vi "Reverse_PolarityTest.vi"(8 "error in (no error)":errorcluster) -> (0 "error out":errorcluster)   [LabVIEW 2025]
uses:
  SubVIs/All test cluster.ctl
  SubVIs/All_enum_ctl.ctl
  SubVIs/Arduino_lamps.ctl
  SubVIs/Lamps_global.vi
  <vilib>/Utility/file.llb/Write Delimited Spreadsheet (string).vi
  <instrlib>/BK Precision 9200 Series/BK Precision 9200 Series.lvlib
  <instrlib>/Keithley 2260B/Keithley 2260B.lvlib
panel:
  out "Table 2":string[][](table)
  in  "ESP PORT":refnum<visa-resource-name>
  out "Connected? 2":bool caption="Long Blank Button"
  out "Tick Time(s)":dbl
  out "Status":string
  in  "POWER SUPPLY":bool caption="Blank Button"
  out "Text name":string
  in  "COM PORT:":refnum<visa-resource-name>
  in  "Start/Stop":bool caption="Slide Switch"
  in  "File Path:":path
  in  "FILENAME":string
  out "Table":string[][](table)
  out "Connected?":bool caption="Long Blank Button"
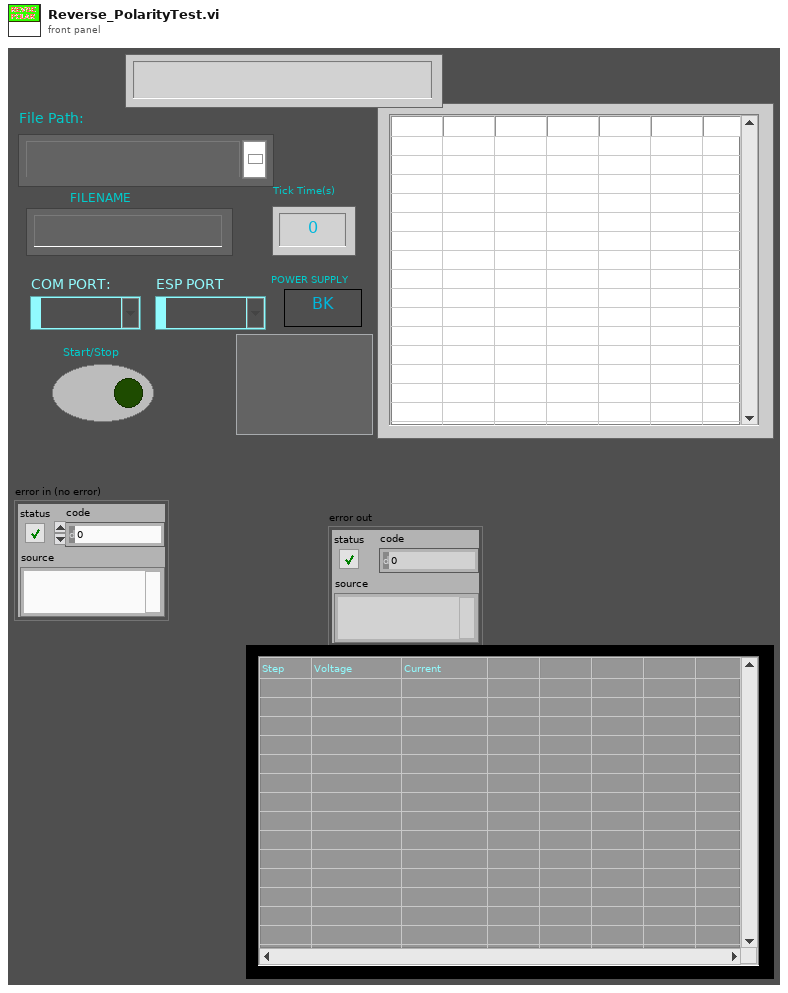
[diagram p1: front panel]
types:
  T1 = enum32{"Invalid", "Standard", "Closed", "Hidden", "Minimized", "Maximized"}
  T2 = typedef "All_enum_ctl.ctl" = enum16{"Init", "Poll", "Connect_esp32", "Connect", "check_start", "Start", "Set_Voltage", "On_relay", "Read_Voltage", "Off_Relay", "Next_Relay", "Next_Step", "Stop", "Store", "Error", "Exit"}
  T3 = typedef "All test cluster.ctl" = cluster{"FilePath":path, "Test Status":bool, "Start Volt":dbl, "End Volt":dbl, "Present Step":dbl, "Present Time(s)":dbl, "End Time":dbl, "Table":string[], "Intensity":string, "BK/Keith":bool, "COM":refnum<visa-resource-name>, "Next state":T2, "Step no.":dbl, "Start ms":u32, "ESP_COM":refnum<visa-resource-name>, "Relay_no":dbl, "Datas":string[]}
  T4 = typedef "Arduino_lamps.ctl" = enum16{"Init", "Poll", "Read", "Write", "Exit"}
  T5 = cluster{"Baud Rate":u32, "Parity":u16, "Data Bits":u16, "Stop Bits":u16, "Flow Control":u16}
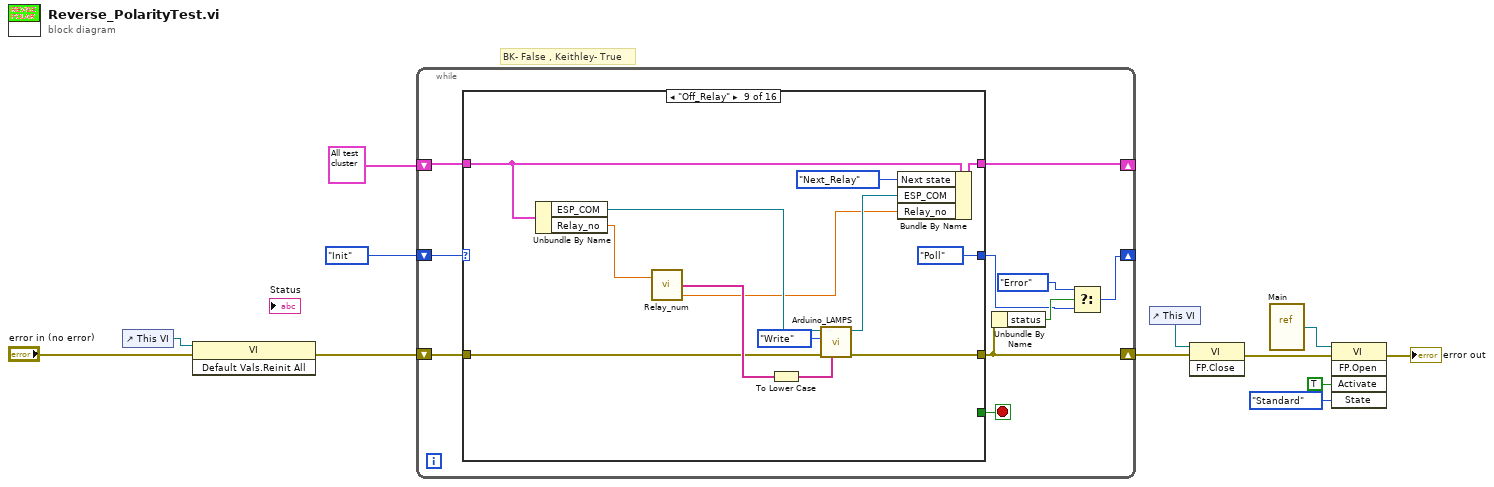
[diagram p0: block diagram]
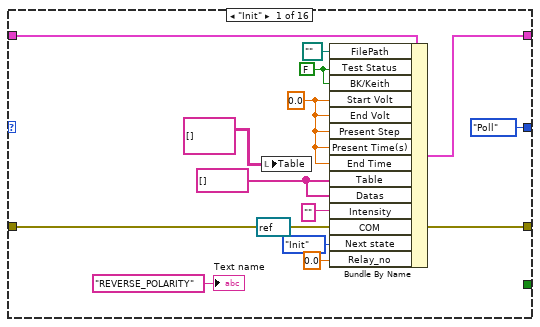
[diagram p2: hidden frame]
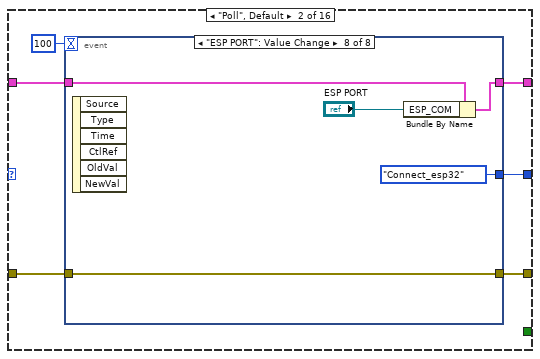
[diagram p3: hidden frame]
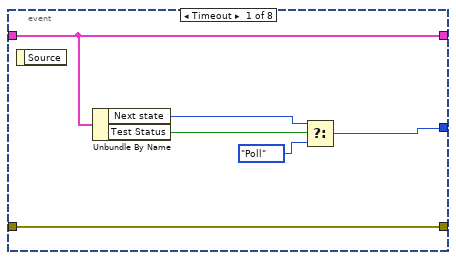
[diagram p4: hidden frame]
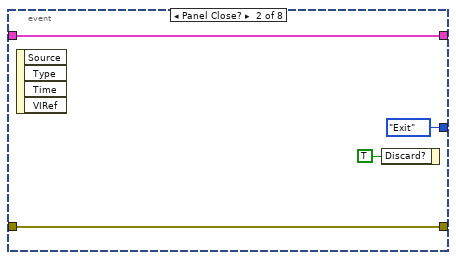
[diagram p5: hidden frame]
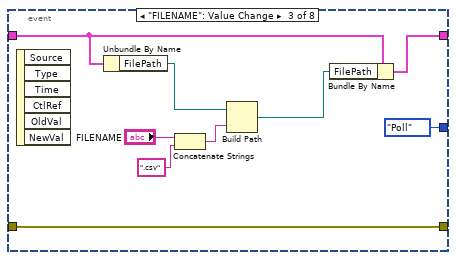
[diagram p6: hidden frame]
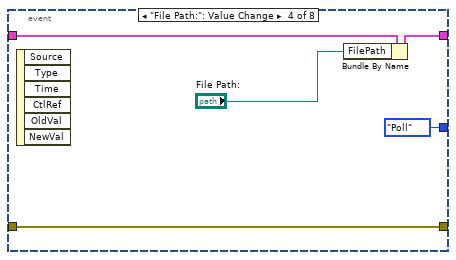
[diagram p7: hidden frame]
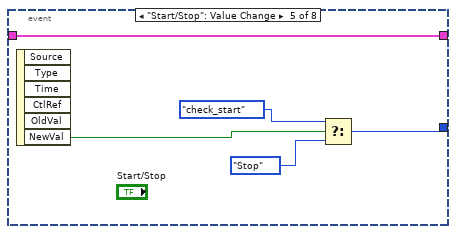
[diagram p8: hidden frame]
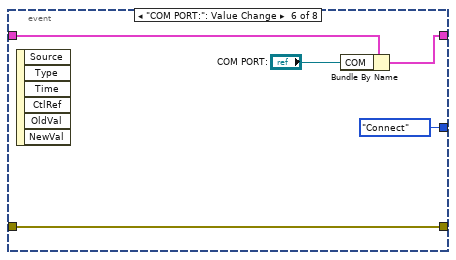
[diagram p9: hidden frame]
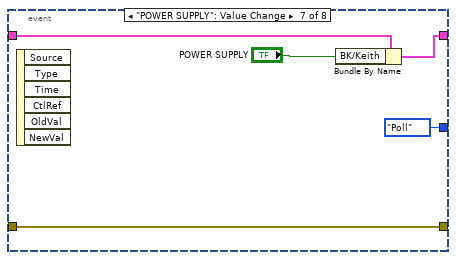
[diagram p10: hidden frame]
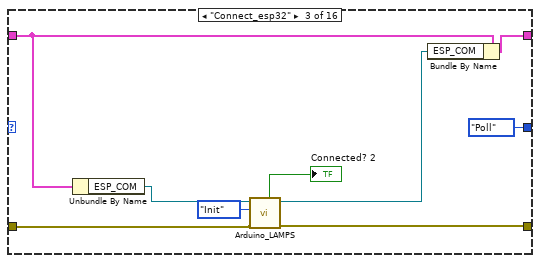
[diagram p11: hidden frame]
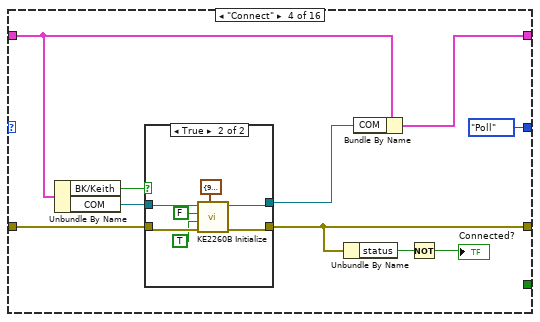
[diagram p12: hidden frame]
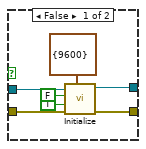
[diagram p13: hidden frame]
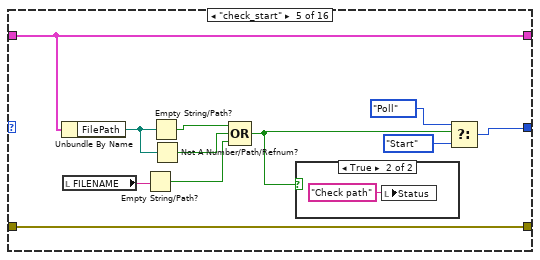
[diagram p14: hidden frame]
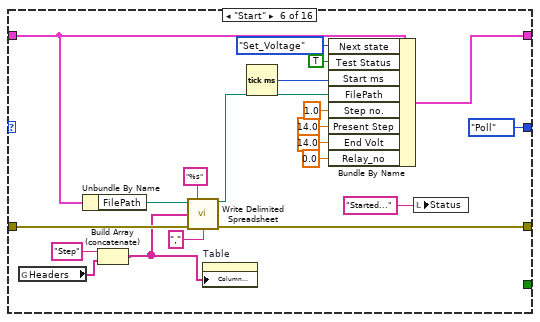
[diagram p16: hidden frame]
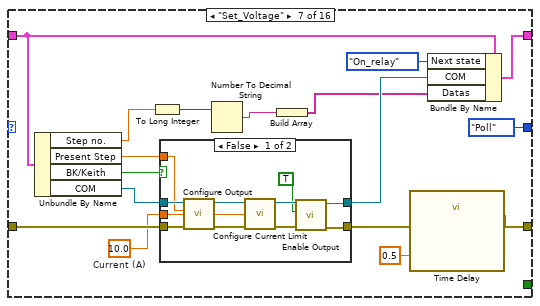
[diagram p17: hidden frame]
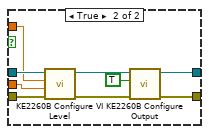
[diagram p18: hidden frame]
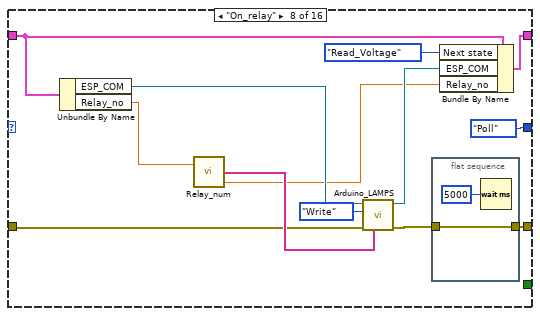
[diagram p19: hidden frame]
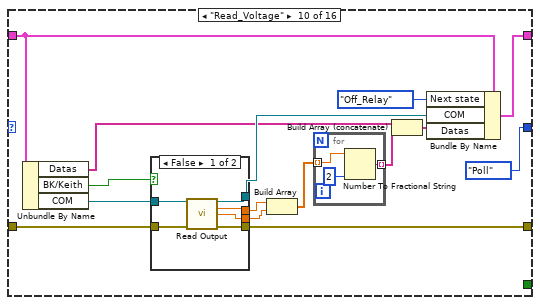
[diagram p20: hidden frame]
diagram:
  # "BK- False , Keithley- True"
  n1 = control-ref of="This VI"() -> (w12:refnum<vi>)
  n2 = invoke class="VI" method="Default Vals.Reinit All"(reference=w12, error in="error in (no error)") -> (error out=w10:errorcluster)  [unwired: 1 in, 2 out]
  n3 = while {
    shift-right: [w21] -> _
    shift-left: T3 {"FilePath"=path "", "Test Status"=FALSE, "Start Volt"=0.0, "End Volt"=0.0, "Present Step"=0.0, "Present Time(s)"=0.0, "End Time"=0.0, "Table"=[], "Intensity"="", "BK/Keith"=FALSE, "COM"="", "Next state"=enum."Init", "Step no."=0.0, "Start ms"=0, "ESP_COM"="", "Relay_no"=0.0, "Datas"=[]} -> [w20]
    shift-right: [w17] -> w2
    shift-left: w10 -> [w19]
    shift-right: [w13] -> _
    shift-left: All_enum_ctl."Init" -> [w22]
    stop <- w18 stop-if-true
    n4 = case shown="\"Off_Relay\"" w22 {
      tunnel: [w34 w39 w88 w97 w129 w150 w167 w189 w205 w226 w256 w262 w293 w315 w356 w376] -> w21
      tunnel: w20 -> [w36 w40 w89 w101 w129 w145 w166 w193 w206 w230 w259 w263 w289 w316 w359 w376]
      tunnel: w19 -> [w35 w42 w93 w105 w130 w147 w168 w192 w209 w231 w260 w268 w288 w320 w363 w381]
      tunnel: [w35 w41 w92 w100 w130 w146 w157 w191 w208 w229 w253 w268 w287 w320 w361 w377] -> w17
      tunnel: [All_enum_ctl."Poll" w37 All_enum_ctl."Poll" All_enum_ctl."Poll" w121 All_enum_ctl."Poll" All_enum_ctl."Poll" All_enum_ctl."Poll" All_enum_ctl."Poll" All_enum_ctl."Poll" All_enum_ctl."Poll" All_enum_ctl."Poll" All_enum_ctl."Poll" All_enum_ctl."Poll" All_enum_ctl."Poll" All_enum_ctl."Exit"] -> w14
      tunnel: [_ _ _ _ _ _ _ _ _ _ _ _ _ _ _ TRUE] -> w18
      frame "Init" {
        w24 = string[] [] ("Table")
        w32 = 0.0 ("Start Volt")
        w30 = FALSE ("Test Status")
        n5 = local write "Table"(string[][] [] ("Table")) -> ()
        n6 = Bundle By Name(cluster=w36, "FilePath"=path "", "Test Status"=w30, "BK/Keith"=w30, "Start Volt"=w32, "End Volt"=w32, "Present Step"=w32, "Present Time(s)"=w32, "End Time"=w32, "Table"=w24, "Datas"=w24, "Intensity"="", "COM"=refnum<visa-resource-name> refnum, "Next state"=All_enum_ctl."Init" ("Last state"), "Relay_no"=0.0) -> (w34:T3)
        "Text name" <- "REVERSE_POLARITY" ("Text name")
      }
      frame "Poll", Default {
        n7 = event shown="[7] \"ESP PORT\": Value Change" {
          selector: _ -> [_ _ _ _ _ _ _ _]
          dyn-events: _ -> [_ _ _ _ _ _ _ _]
          timeout: 100 -> [_ _ _ _ _ _ _ _]
          tunnel: w42 -> [w48 w49 w61 w64 _ w72 w77 w83]
          tunnel: [w48 w49 w61 w64 _ w72 w77 w83] -> w41
          tunnel: w40 -> [w47 w50 w59 w66 w70 w76 w81 w86]
          tunnel: [w47 w50 w55 w63 w70 w75 w80 w85] -> w39
          tunnel: [w43 All_enum_ctl."Exit" ("f") All_enum_ctl."Poll" All_enum_ctl."Poll" w67 All_enum_ctl."Connect" ("f") All_enum_ctl."Poll" ("f") All_enum_ctl."Connect_esp32" ("f")] -> w37
          event Timeout {
            n8 = event-data() -> ()  [unwired: 1 in, 1 out]
            n9 = Unbundle By Name(w47) -> ("Next state"=w44:T2, "Test Status"=w46:bool)
            n10 = Select(t=w44, s=w46, f=All_enum_ctl."Poll") -> (s? t:f=w43:T2)
          }
          event Panel Close? {
            n11 = event-data() -> ()  [unwired: 1 in, 4 out]
            n12 = event-data("Discard?"=TRUE) -> ()  [unwired: 1 in, 1 out]
          }
          event "FILENAME": Value Change {
            n13 = event-data() -> ()  [unwired: 1 in, 6 out]
            n14 = Unbundle By Name(w59) -> ("FilePath"=w58:path)
            n15 = Concatenate Strings("FILENAME", ".csv" ("string")) -> (w57:string)
            n16 = Build Path(base path=w58, name or relative path=w57) -> (appended path=w54:path)
            n17 = Bundle By Name(cluster=w59, "FilePath"=w54) -> (w55:T3)
          }
          event "File Path:": Value Change {
            n18 = event-data() -> ()  [unwired: 1 in, 6 out]
            n19 = Bundle By Name(cluster=w66, "FilePath"="File Path:") -> (w63:T3)
          }
          event "Start/Stop": Value Change {
            n20 = event-data() -> ("NewVal"=w71:bool)  [unwired: 1 in, 5 out]
            n21 = Select(t=All_enum_ctl."check_start", s=w71, f=All_enum_ctl."Stop") -> (s? t:f=w67:T2)
          }
          event "COM PORT:": Value Change {
            n22 = event-data() -> ()  [unwired: 1 in, 6 out]
            n23 = Bundle By Name(cluster=w76, "COM"="COM PORT:") -> (w75:T3)
          }
          event "POWER SUPPLY": Value Change {
            n24 = event-data() -> ()  [unwired: 1 in, 6 out]
            n25 = Bundle By Name(cluster=w81, "BK/Keith"="POWER SUPPLY") -> (w80:T3)
          }
          event "ESP PORT": Value Change {
            n26 = event-data() -> ()  [unwired: 1 in, 6 out]
            n27 = Bundle By Name(cluster=w86, "ESP_COM"="ESP PORT") -> (w85:T3)
          }
        }
      }
      frame "Connect_esp32" {
        n28 = Unbundle By Name(w89) -> ("ESP_COM"=w95:refnum<visa-resource-name>)
        n29 = call "Arduino_LAMPS.vi"("error out"=w93, "Enum"=Arduino_lamps."Init", "VISA resource name"=w95) -> ("error out 2"=w92:errorcluster, "VISA out"=w87:refnum<visa-resource-name>, "status"=→"Connected? 2":bool)  [unwired: 4 in, 2 out]
        n30 = Bundle By Name(cluster=w89, "ESP_COM"=w87) -> (w88:T3)
      }
      frame "Connect" {
        n31 = Unbundle By Name(w101) -> ("BK/Keith"=w99:bool, "COM"=w98:refnum<visa-resource-name>)
        n32 = case shown="True" w99 {
          tunnel: w105 -> [w112 w119]
          tunnel: [w111 w118] -> w100
          tunnel: w98 -> [w110 w117]
          tunnel: [w106 w115] -> w96
          frame False {
            n33 = call <instrlib>:"Initialize.vi"("Serial Configuration"=cluster{"Baud Rate":u32} {"Baud Rate"=9600}, "error in (no error)"=w112, "Reset (True)"=TRUE, "ID Query (True)"=FALSE, "VISA resource name"=w110) -> ("error out"=w111:errorcluster, "VISA resource name out"=w106:refnum<visa-resource-name>)  [unwired: 5 in]
          }
          frame True {
            n34 = call <instrlib>:"KE2260B Initialize.vi"("Serial Configuration"=T5 {"Baud Rate"=9600, "Parity"=0, "Data Bits"=8, "Stop Bits"=10, "Flow Control"=0}, "error in (no error)"=w119, "Reset (True)"=TRUE, "ID Query (True)"=FALSE, "VISA resource name"=w117) -> ("error out"=w118:errorcluster, "VISA resource name out"=w115:refnum<visa-resource-name>)  [unwired: 5 in]
          }
        }
        n35 = Unbundle By Name(w100) -> ("status"=w104:bool)
        n36 = Bundle By Name(cluster=w101, "COM"=w96) -> (w97:T3)
        n37 = Not(x=w104) -> (.not. x?=→"Connected?":bool)
      }
      frame "check_start" {
        n38 = Unbundle By Name(w129) -> ("FilePath"=w127:path)
        n39 = local read "FILENAME"() -> (w128:string)
        n40 = Empty String/Path?(string/path=w128) -> (empty?=w124:bool)
        n41 = Empty String/Path?(string/path=w127) -> (empty?=w126:bool)
        n42 = Not A Number/Path/Refnum?(number/path/refnum=w127) -> (NaN/Path/Refnum?=w125:bool)
        n43 = Compound Arithmetic op=OR(w126, w125, w124) -> (w120:bool)
        n44 = case shown="True" w120 {
          frame False {
          }
          frame True {
            n45 = local write "Status"("Check path") -> ()
          }
        }
        n46 = Select(t=All_enum_ctl."Poll", s=w120, f=All_enum_ctl."Start") -> (s? t:f=w121:T2)
      }
      frame "Start" {
        n47 = global read "Lamps_global.vi" "Headers"() -> (w135:string[])
        n48 = Unbundle By Name(w145) -> ("FilePath"=w144:path)
        n49 = Build Array (concatenate)("Step" ("String"), w135) -> (w133:string[])
        n50 = call-poly <vilib>:"Write Delimited Spreadsheet.vi"("file path (dialog if empty)"=w144, "format (%s)"="%s" ("format (%.3f)"), "1D data"=w133, "error in (no error)"=w147, "delimiter (\\t)"="," ("delimiter (\\t)")) -> ("new file path (Not A Path if cancelled)"=w141:path, "error out"=w146:errorcluster)  [unwired: 9 in]
        n51 = property on="Table" class="Tbl (strict)"("Column Headers[]"=w133) -> ()  [unwired: 2 in, 2 out]
        n52 = Tick Count (ms)() -> (millisecond timer value=w139:u32)
        n53 = Bundle By Name(cluster=w145, "Next state"=All_enum_ctl."Set_Voltage" ("Last state"), "Test Status"=TRUE, "Start ms"=w139, "FilePath"=w141, "Step no."=1.0, "Present Step"=14.0, "End Volt"=14.0, "Relay_no"=0.0) -> (w150:T3)
        n54 = local write "Status"("Started...") -> ()
      }
      frame "Set_Voltage" {
        w159 = 10.0  # Current (A)
        n55 = Unbundle By Name(w166) -> ("Step no."=w153:dbl, "Present Step"=w160:dbl, "BK/Keith"=w161:bool, "COM"=w164:refnum<visa-resource-name>)
        n56 = To Long Integer(number=w153) -> (32bit integer=w155:i32)
        n57 = case shown="False" w161 {
          tunnel: w168 -> [w172 w188]
          tunnel: [w179 w187] -> w165
          tunnel: w164 -> [w177 w185]
          tunnel: [w178 w183] -> w163
          tunnel: w160 -> [w176 w181]
          tunnel: w159 -> [w170 w180]
          frame False {
            n58 = call <instrlib>:"Configure Output.vi"("error in (no error)"=w172, "Voltage Level (0.0 V)"=w176, "VISA resource name"=w177) -> ("error out"=w173:errorcluster, "VISA resource name out"=w171:refnum<visa-resource-name>)  [unwired: 7 in]
            n59 = call <instrlib>:"Configure Current Limit.vi"("error in (no error)"=w173, "Current Limit (0.0 A)"=w170, "VISA resource name"=w171) -> ("error out"=w175:errorcluster, "VISA resource name out"=w174:refnum<visa-resource-name>)  [unwired: 7 in]
            n60 = call <instrlib>:"Enable Output.vi"("error in (no error)"=w175, "Enable Output (F: False)"=TRUE, "VISA resource name"=w174) -> ("error out"=w179:errorcluster, "VISA resource name out"=w178:refnum<visa-resource-name>)  [unwired: 7 in]
          }
          frame True {
            n61 = call <instrlib>:"KE2260B Configure VI Level.vi"("error in (no error)"=w188, "Current Level (0.000 A)"=w180, "Voltage Level (0.000 V)"=w181, "VISA resource name"=w185) -> ("error out"=w186:errorcluster, "VISA resource name out"=w184:refnum<visa-resource-name>)  [unwired: 6 in]
            n62 = call <instrlib>:"KE2260B Configure Output.vi"("error in (no error)"=w186, "Enable Output (T: Enable)"=TRUE, "VISA resource name"=w184) -> ("error out"=w187:errorcluster, "VISA resource name out"=w183:refnum<visa-resource-name>)  [unwired: 7 in]
          }
        }
        n63 = Number To Decimal String(number=w155) -> (decimal integer string=w154:string)  [unwired: 1 in]
        n64 = Build Array(w154) -> (w152:string[])
        n65 = call "Time Delay"("error in (no error)"=w165, "Delay Time (s)"=0.5) -> ("error out"=w157:errorcluster)  [unwired: 9 in]
        n66 = Bundle By Name(cluster=w166, "Next state"=All_enum_ctl."On_relay", "COM"=w163, "Datas"=w152) -> (w167:T3)
      }
      frame "On_relay" {
        n67 = Unbundle By Name(w193) -> ("ESP_COM"=w201:refnum<visa-resource-name>, "Relay_no"=w196:dbl)
        n68 = call "Relay_num.vi"("Relay_no."=w196) -> ("Relay"=w195:string[], "Relay_no.out"=w194:dbl)  [unwired: 1 in, 1 out]
        n69 = call "Arduino_LAMPS.vi"("DO's"=w195, "error out"=w192, "Enum"=Arduino_lamps."Write", "VISA resource name"=w201) -> ("error out 2"=w197:errorcluster, "VISA out"=w199:refnum<visa-resource-name>)  [unwired: 3 in, 3 out]
        n70 = flat-sequence {
          tunnel: w197 -> [w203]
          tunnel: [w203] -> w191
          frame #0 {
            n71 = Wait (ms)(milliseconds to wait=u32 5000) -> ()  [unwired: 1 out]
          }
        }
        n72 = Bundle By Name(cluster=w193, "Next state"=All_enum_ctl."Read_Voltage", "ESP_COM"=w199, "Relay_no"=w194) -> (w189:T3)
      }
      frame "Off_Relay" {
        n73 = Unbundle By Name(w206) -> ("ESP_COM"=w216:refnum<visa-resource-name>, "Relay_no"=w212:dbl)
        n74 = call "Relay_num.vi"("Relay_no."=w212) -> ("Relay"=w211:string[], "Relay_no.out"=w210:dbl)  [unwired: 1 in, 1 out]
        n75 = To Lower Case(string=w211) -> (all lower case string=w204:string[])
        n76 = call "Arduino_LAMPS.vi"("DO's"=w204, "error out"=w209, "Enum"=Arduino_lamps."Write", "VISA resource name"=w216) -> ("error out 2"=w208:errorcluster, "VISA out"=w214:refnum<visa-resource-name>)  [unwired: 3 in, 3 out]
        n77 = Bundle By Name(cluster=w206, "Next state"=All_enum_ctl."Next_Relay", "ESP_COM"=w214, "Relay_no"=w210) -> (w205:T3)
      }
      frame "Read_Voltage" {
        n78 = Unbundle By Name(w230) -> ("Datas"=w217:string[], "BK/Keith"=w227:bool, "COM"=w228:refnum<visa-resource-name>)
        n79 = case shown="False" w227 {
          tunnel: w231 -> [w237 w243]
          tunnel: [w236 w242] -> w229
          tunnel: w228 -> [w235 w240]
          tunnel: [w234 w241] -> w225
          tunnel: [w233 w239] -> w222
          tunnel: [w232 w238] -> w221
          frame False {
            n80 = call <instrlib>:"Read Output.vi"("VISA resource name"=w235, "error in (no error)"=w237) -> ("VISA resource name out"=w234:refnum<visa-resource-name>, "Actual Voltage Level (V)"=w233:dbl, "Actual Current Level (A)"=w232:dbl, "error out"=w236:errorcluster)  [unwired: 9 in, 1 out]
          }
          frame True {
            n81 = call <instrlib>:"KE2260B Read Output.vi"("error in (no error)"=w243, "VISA resource name"=w240) -> ("error out"=w242:errorcluster, "Actual Current Level (A)"=w238:dbl, "Actual Voltage Level (V)"=w239:dbl, "VISA resource name out"=w241:refnum<visa-resource-name>)  [unwired: 6 in]
          }
        }
        n82 = Build Array(w222, w221) -> (w220:dbl[])
        n83 = for {
          tunnel: w220 -> [w245] mode=indexing
          tunnel: [w244] -> w219 mode=indexing
          n84 = Number To Fractional String(number=w245, precision (6)=i16 2) -> (F-format string=w244:string)  [unwired: 2 in]
        }
        n85 = Build Array (concatenate)(w217, w219) -> (w218:string[])
        n86 = Bundle By Name(cluster=w230, "Next state"=All_enum_ctl."Off_Relay", "COM"=w225, "Datas"=w218) -> (w226:T3)
      }
      frame "Store" {
        n87 = Unbundle By Name(w259) -> ("Table"=w250:string[], "FilePath"=w252:path)
        n88 = local read "Table"() -> (w258:string[][])
        n89 = Build Array (concatenate)(w258, w250) -> (→"Table":string[][])
        n90 = call-poly <vilib>:"Write Delimited Spreadsheet.vi"("file path (dialog if empty)"=w252, "format (%s)"="%s", "1D data"=w250, "append to file? (new file:F)"=TRUE, "error in (no error)"=w260, "delimiter (\\t)"="," ("delimiter (\\t)")) -> ("new file path (Not A Path if cancelled)"=w249:path, "error out"=w253:errorcluster)  [unwired: 8 in]
        n91 = Bundle By Name(cluster=w259, "Next state"=All_enum_ctl."Next_Step", "FilePath"=w249) -> (w256:T3)
      }
      frame "Next_Relay" {
        n92 = Unbundle By Name(w263) -> ("Relay_no"=w267:dbl, "Datas"=w264:string[])
        n93 = call "Relay_num.vi"("Relay_no."=w267) -> ("x = y?"=w266:bool, "Relay_no.out"=w265:dbl)  [unwired: 1 in, 1 out]
        n94 = case shown="True" w266 {
          tunnel: [w278 w283] -> w262
          tunnel: w263 -> [w277 w282]
          tunnel: w265 -> [w275 _]
          tunnel: w264 -> [w269 w279]
          frame False {
            n95 = local read "Table 2"() -> (w273:string[][])
            n96 = Increment(x=w275) -> (x+1=w274:dbl)
            n97 = Array Size(array=w273) -> (size(s)=w271:i32[])
            n98 = Index Array(array=w271) -> (element=w270:i32)  [unwired: 1 in]
            n99 = Bundle By Name(cluster=w277, "Next state"=All_enum_ctl."On_relay", "Relay_no"=w274, "Datas"=w269) -> (w278:T3)
            n100 = Replace Array Subset(array=w273, new element=w269, index (row)=w270) -> (w272:string[][])  [unwired: 1 in]
            n101 = local write "Table 2"(w272) -> ()
          }
          frame True {
            n102 = Bundle By Name(cluster=w282, "Next state"=All_enum_ctl."Store", "Relay_no"=0.0, "Table"=w279) -> (w283:T3)
          }
        }
      }
      frame "Stop" {
        n103 = Unbundle By Name(w289) -> ("BK/Keith"=w290:bool, "COM"=w291:refnum<visa-resource-name>)
        n104 = case shown="False" w290 {
          tunnel: w288 -> [w297 w303]
          tunnel: [w299 w304] -> w287
          tunnel: w291 -> [w296 w302]
          tunnel: [w298 w301] -> w286
          frame False {
            n105 = call <instrlib>:"Enable Output.vi"("error in (no error)"=w297, "Enable Output (F: False)"=FALSE, "VISA resource name"=w296) -> ("error out"=w299:errorcluster, "VISA resource name out"=w298:refnum<visa-resource-name>)  [unwired: 7 in]
          }
          frame True {
            n106 = call <instrlib>:"KE2260B Configure Output.vi"("error in (no error)"=w303, "Enable Output (T: Enable)"=FALSE, "VISA resource name"=w302) -> ("error out"=w304:errorcluster, "VISA resource name out"=w301:refnum<visa-resource-name>)  [unwired: 7 in]
          }
        }
        n107 = local write "Start/Stop"(FALSE) -> ()
        n108 = Bundle By Name(cluster=w289, "Test Status"=FALSE, "COM"=w286) -> (w293:T3)
        n109 = local write "Status"("Test Stopped....") -> ()
      }
      frame "Next_Step" {
        n110 = Unbundle By Name(w316) -> ("Start ms"=w312:u32, "Present Step"=w317:dbl, "End Volt"=w318:dbl, "Step no."=w313:dbl)
        n111 = Tick Count (ms)() -> (millisecond timer value=w306:u32)
        n112 = Subtract(x=w306, y=w312) -> (x-y=w311:u32)
        n113 = Equal?(x=w317, y=w318) -> (x = y?=w319:bool)
        n114 = Divide(x=w311, y=u32 1000) -> (x/y=w309:dbl)
        n115 = To Unsigned Word Integer(number=w309) -> (unsigned 16bit integer=w305:u16)
        "Tick Time(s)" <- w305
        n116 = Greater Or Equal?(x=w305, y=u16 60) -> (x >= y?=w307:bool)
        n117 = case shown="True" w319 {
          tunnel: w317 -> [w322 w341]
          tunnel: w316 -> [w329 w345]
          tunnel: [w328 w344] -> w315
          tunnel: w313 -> [w326 w342]
          tunnel: w307 -> [w324 w343]
          tunnel: w306 -> [w323 _]
          frame False {
            n118 = Increment(x=w326) -> (x+1=w325:dbl)
            n119 = case shown="True" w324 {
              tunnel: w329 -> [w334 w340]
              tunnel: [w333 w339] -> w328
              tunnel: All_enum_ctl."Set_Voltage" ("Next state") -> [w332 w338]
              tunnel: w325 -> [w331 w337]
              tunnel: w322 -> [w330 _]
              tunnel: w323 -> [_ w336]
              tunnel: 24.0 ("Present Step") -> [_ w335]
              frame False {
                n120 = Bundle By Name(cluster=w334, "Next state"=w332, "Present Step"=w330, "Step no."=w331) -> (w333:T3)
              }
              frame True {
                n121 = Bundle By Name(cluster=w340, "Start ms"=w336, "Next state"=w338, "Present Step"=w335, "Step no."=w337) -> (w339:T3)
              }
            }
          }
          frame True {
            n122 = case shown="False" w343 {
              tunnel: w345 -> [w348 w354]
              tunnel: [w347 w353] -> w344
              tunnel: w342 -> [w350 _]
              tunnel: w341 -> [w346 _]
              frame False {
                n123 = Increment(x=w350) -> (x+1=w349:dbl)
                n124 = Bundle By Name(cluster=w348, "Next state"=All_enum_ctl."Set_Voltage", "Present Step"=w346, "Step no."=w349) -> (w347:T3)
              }
              frame True {
                n125 = Bundle By Name(cluster=w354, "Next state"=All_enum_ctl."Stop") -> (w353:T3)
              }
            }
          }
        }
      }
      frame "Error" {
        n126 = Unbundle By Name(w359) -> ("BK/Keith"=w357:bool, "COM"=w358:refnum<visa-resource-name>)
        n127 = case shown="False" w357 {
          tunnel: w363 -> [w366 w371]
          tunnel: [w367 w370] -> w360
          tunnel: w358 -> [w365 w369]
          tunnel: [w364 w368] -> w355
          frame False {
            n128 = call <instrlib>:"Reset.vi"("error in (no error)"=w366, "VISA resource name"=w365) -> ("error out"=w367:errorcluster, "VISA resource name out"=w364:refnum<visa-resource-name>)  [unwired: 8 in]
          }
          frame True {
            n129 = call <instrlib>:"KE2260B Reset.vi"("error in (no error)"=w371, "VISA resource name"=w369) -> ("error out"=w370:errorcluster, "VISA resource name out"=w368:refnum<visa-resource-name>)  [unwired: 8 in]
          }
        }
        n130 = call <vilib>:"Clear Errors.vi"("error in (no error)"=w360) -> ("error out"=w361:errorcluster)  [unwired: 5 in, 1 out]
        n131 = Bundle By Name(cluster=w359, "COM"=w355) -> (w356:T3)
      }
      frame "Exit" {
        n132 = Unbundle By Name(w376) -> ("ESP_COM"=w372:refnum<visa-resource-name>, "BK/Keith"=w374:bool, "COM"=w375:refnum<visa-resource-name>)
        n133 = case shown="False" w374 {
          tunnel: w381 -> [w384 w387]
          tunnel: [w383 w386] -> w378
          tunnel: w375 -> [w382 w385]
          frame False {
            n134 = call <instrlib>:"Close.vi"("error in (no error)"=w384, "VISA resource name"=w382) -> ("error out"=w383:errorcluster)  [unwired: 9 in]
          }
          frame True {
            n135 = call <instrlib>:"KE2260B Close.vi"("error in (no error)"=w387, "VISA resource name"=w385) -> ("error out"=w386:errorcluster)  [unwired: 9 in]
          }
        }
        n136 = VISA Close(VISA resource name=w372, error in (no error)=w378) -> (error out=w373:errorcluster)
        n137 = call <vilib>:"Clear Errors.vi"("error in (no error)"=w373) -> ("error out"=w377:errorcluster)  [unwired: 5 in, 1 out]
      }
    }
    n138 = Unbundle By Name(w17) -> ("status"=w16:bool)
    n139 = Select(t=All_enum_ctl."Error", s=w16, f=w14) -> (s? t:f=w13:T2)
  }
  n140 = control-ref of="This VI"() -> (w3:refnum<vi>)
  n141 = invoke class="VI" method="FP.Close"(reference=w3, error in=w2) -> (error out=w1:errorcluster)  [unwired: 1 in, 2 out]
  n142 = vi-ref "Main.vi"() -> (w7:refnum<vi>)
  n143 = invoke class="VI" method="FP.Open"(reference=w7, error in=w1, "Activate"=TRUE ("Activate?"), "State"=T1."Standard") -> (error out=→"error out":errorcluster)  [unwired: 1 in, 4 out]
